vi "WriteDO.vi"(8 "error in (no error)":errorcluster, 9 "DO Value (True)":bool=TRUE, 10 "Output":T1, 11 "VISA resource name":refnum<visa-resource-name>) -> (0 "error out":errorcluster, 3 "VISA resource name out":refnum<visa-resource-name>)   [LabVIEW 2020, in "HandsOnPi2040.lvlib"]
doc: "Establishes communication with the instrument and optionally performs an instrument identification query and/or an instrument reset. It also places the instrument in a default state needed for other instrument driver operations. Therefore, call this VI before calling other instrument driver VIs for this instrument. Generally, you need to call the <b>Initialize</b> VI only once at the beginning of an application."
uses:
  HandsOnPi2040.lvlib
  cti-drivers-lv-visa-main/CTI-Visa/CTI-Visa.lvlib
  DigOuts.ctl
panel:
  # "Output"
  # "Input"
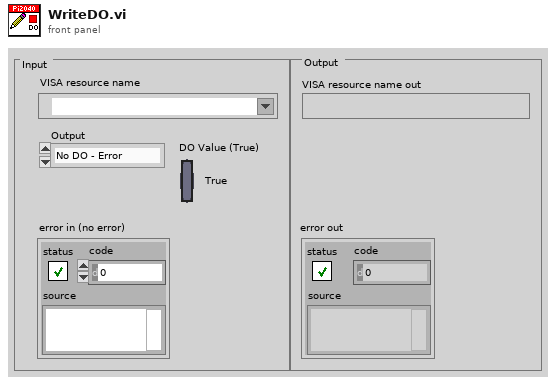
[diagram p1: front panel]
types:
  T1 = typedef "HandsOnPi2040.lvlib/DigOuts.ctl" = enum16{"No DO - Error", "DO1 (GPIO2)", "DO2 (GPIO3)", "DO3 (GPIO4)", "DO4 (GPIO5)", "BEEP (GPIO6)"}
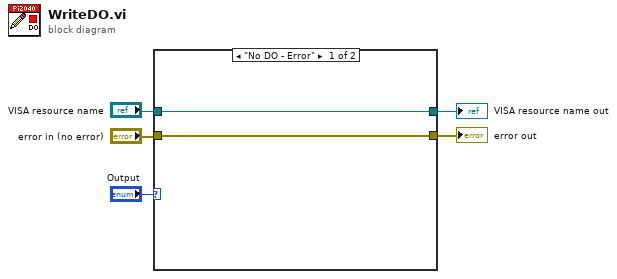
[diagram p0: block diagram]
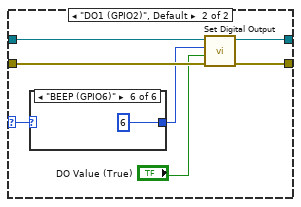
[diagram p2: hidden frame]
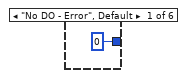
[diagram p3: hidden frame]
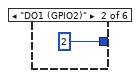
[diagram p4: hidden frame]
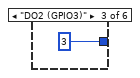
[diagram p5: hidden frame]
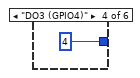
[diagram p6: hidden frame]
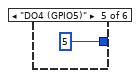
[diagram p7: hidden frame]
diagram:
  n1 = case shown="\"No DO - Error\"" "Output" {
    selector: "Output" -> [_ w14]
    tunnel: [w7 w12] -> w4
    tunnel: [w6 w11] -> w5
    tunnel: "VISA resource name" -> [w6 w10]
    tunnel: "error in (no error)" -> [w7 w13]
    frame "No DO - Error" {
    }
    frame "DO1 (GPIO2)", Default {
      n2 = case shown="\"BEEP (GPIO6)\"" w14 {
        tunnel: [0 2 3 4 5 6] -> w9
        frame "No DO - Error", Default {
        }
        frame "DO1 (GPIO2)" {
        }
        frame "DO2 (GPIO3)" {
        }
        frame "DO3 (GPIO4)" {
        }
        frame "DO4 (GPIO5)" {
        }
        frame "BEEP (GPIO6)" {
        }
      }
      n3 = call "Set Digital Output.vi"("error in (no error)"=w13, "Value"="DO Value (True)", "Channel"=w9, "VISA resource name in"=w10) -> ("error out"=w12:errorcluster, "VISA resource name"=w11:refnum<visa-resource-name>)  [unwired: 6 in]
    }
  }
  "VISA resource name out" <- w5
  "error out" <- w4
